vi "Main.vi"() -> ()   [LabVIEW 2026]
uses:
  <vilib>/Instr/_visa.llb/VISA Configure Serial Port (Instr).vi
panel:
  out "SR MODO":enum16{"AUTOMATICO", "MANUAL"}(ring)=enum."MANUAL"
  out "Boton Reset":string
  out "Errores CRC":dbl
  out "Tramas OK":dbl
  out "Estado":string
  out "SALIDA PWM":dbl(graph)
  in  "MODO":bool=TRUE
  in  "RESET":bool
  out "Maquina":T1(ring)
  in  "EMERGENCIA":bool
  in  "PWM":dbl min=0.0 max=100.0
  out "SP Vs ALTURA":cluster{dbl, dbl}(graph)
  out "PING PONG":dbl(slide) scale=0.0..50.0
  out "PID":T2(ring)
  out "error out":errorcluster
  out "Enum":enum16{"DESCONECTADO", "CONECTADO"}(ring)
  out "ESTADO  SYS":enum16{"DETENIDO", "EJECUTANDO", "ERROR"}(ring)
  in  "PARADA":bool
  in  "INICIO":bool
  out "PID":string
  in  "SP":dbl=25.0 min=0.0 max=100.0
  in  "KD":dbl=0.07 min=0.0 max=65535.0
  in  "KI":dbl=0.14 min=0.0 max=65535.0
  in  "KP":dbl=3.9 min=0.0 max=65535.0
  in  "PID":bool
  out "PWM":dbl format="%.2g"
  out "ERROR":dbl format="%.2g"
  out "ALTURA":dbl format="%.2g"
  out "SP":dbl format="%.2f"
  out "array":string[][](array[string])
  out "Procesar":string
  in  "Stop Simulation":bool
  in  "Numeric":u32=115200
  in  "VISA resource name":refnum<visa-resource-name>="COM12"
  out "Iteracion":i32
  # "Sistema Levitador Neumático"
  # "Planta"
  # "Grafico en Tiempo Real"
  # "COMUNICACIÓN"
  # "ESTADO DEL SISTEMA"
  # "Estado :"
  # "Puerto :"
  # "Comunicación :"
  # "Baud :"
  # "Estado PID :"
  # "CONFIGURACIÓN PID"
  # "VARIABLES EN TIEMPO REAL"
  # "KP :"
  # "KI  :"
  # "KD :"
  # "AUTO"
  # "MANUAL"
  # "SP :"
  # "PWM :"
  # "Mensaje a Procesar :"
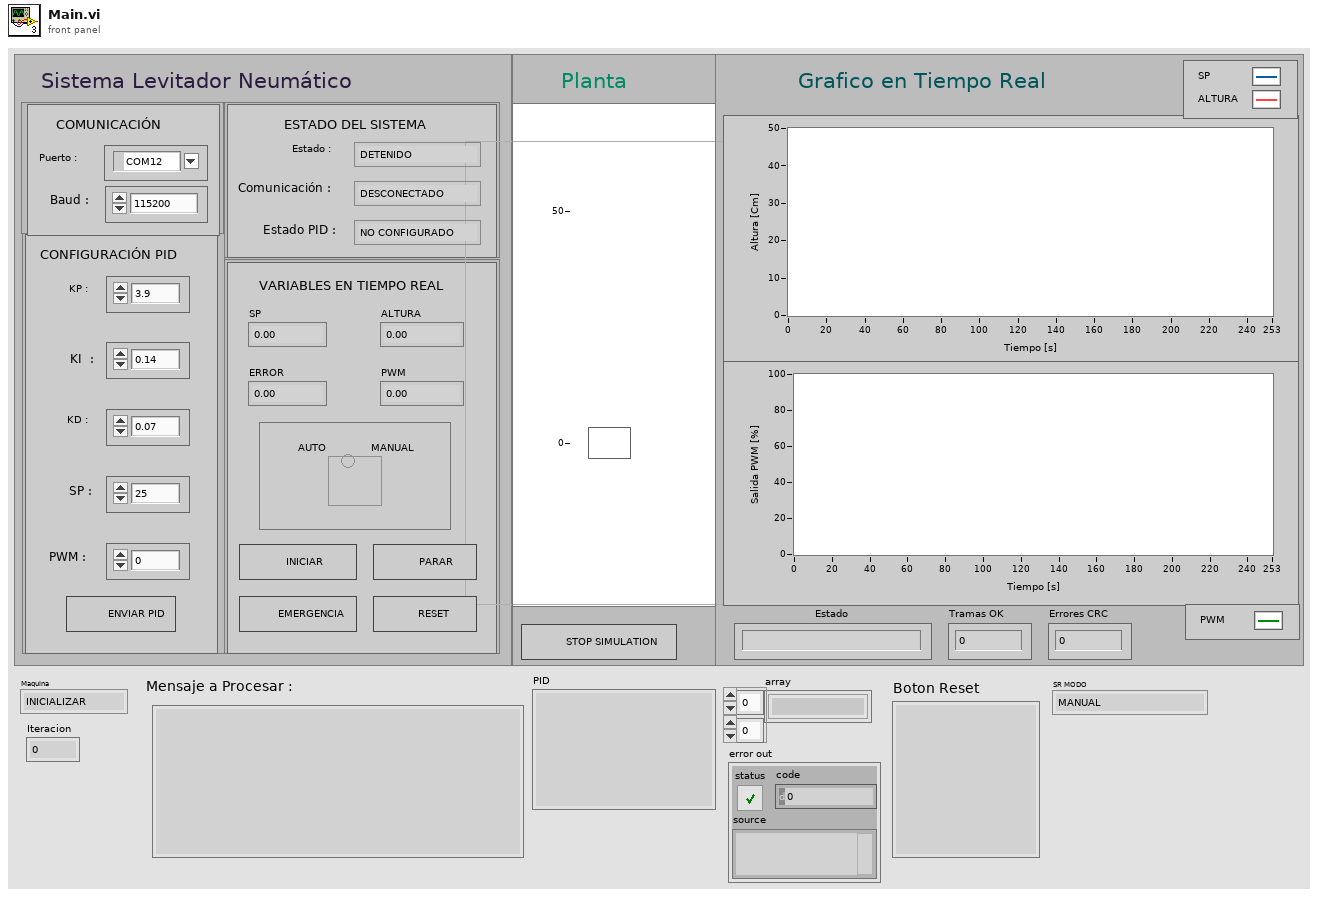
[diagram p1: front panel]
types:
  T1 = enum16{"INICIALIZAR", "ESPERA", "ENVIAR_MODO", "ENVIAR_SP", "ENVIAR_PID", "RECIBIR", "PROCESAR", "ENVIAR_RESET", "ENVIAR_RUN", "ENVIAR_STOP", "ENVIAR_EMERGENCIA_ON", "ENVIAR_EMERGENCIA_OFF", "ERROR", "CERRAR"}
  T2 = enum16{"NO CONFIGURADO", "CONFIGURADO", "AUTOMATICO"}
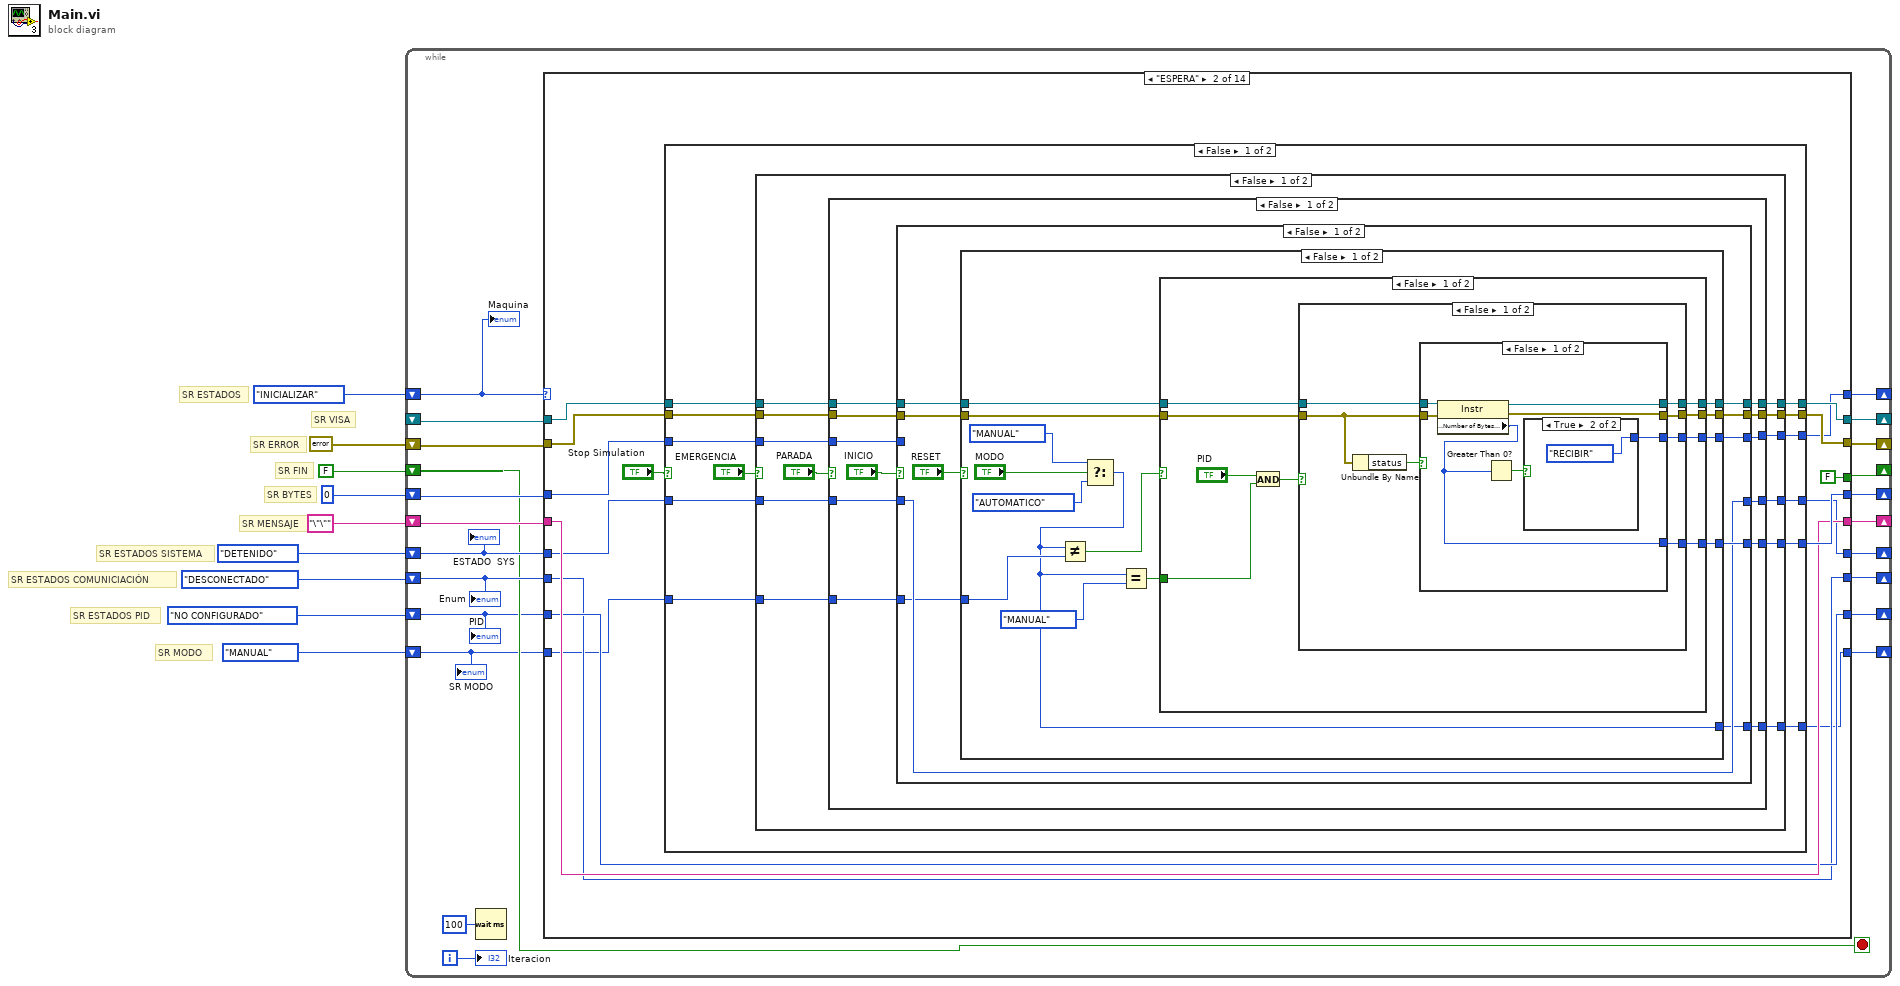
[diagram p0: block diagram]
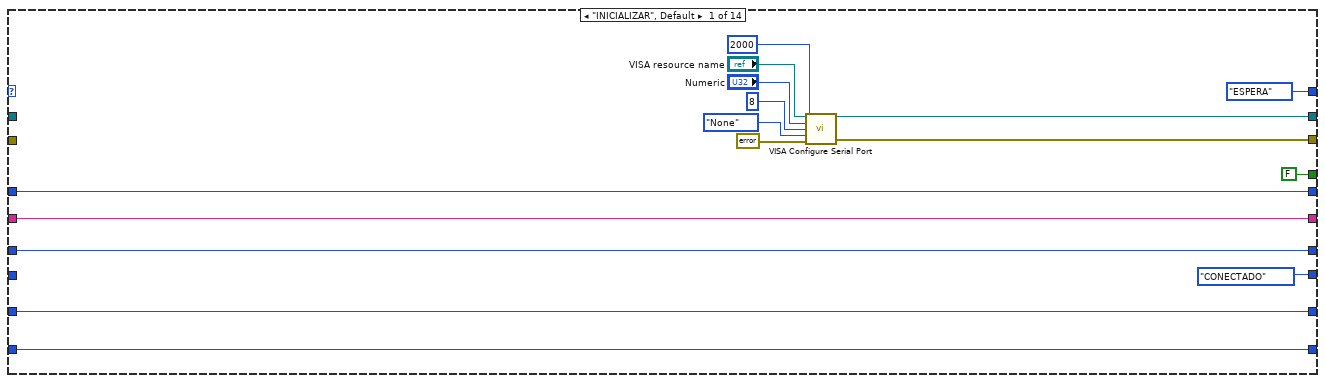
[diagram p2: hidden frame]
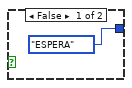
[diagram p3: hidden frame]
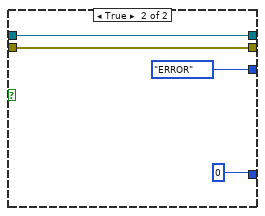
[diagram p4: hidden frame]
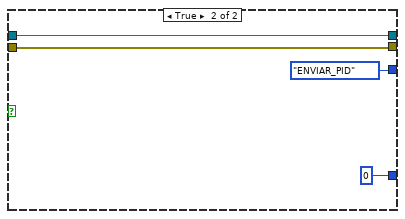
[diagram p5: hidden frame]
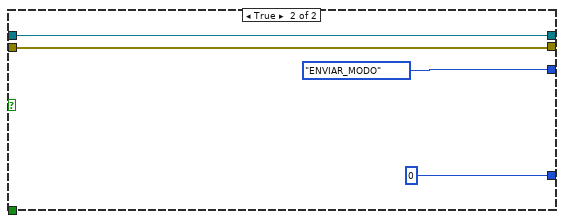
[diagram p6: hidden frame]
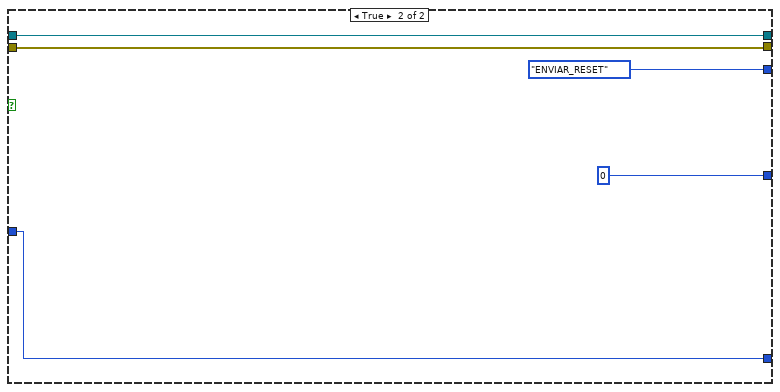
[diagram p7: hidden frame]
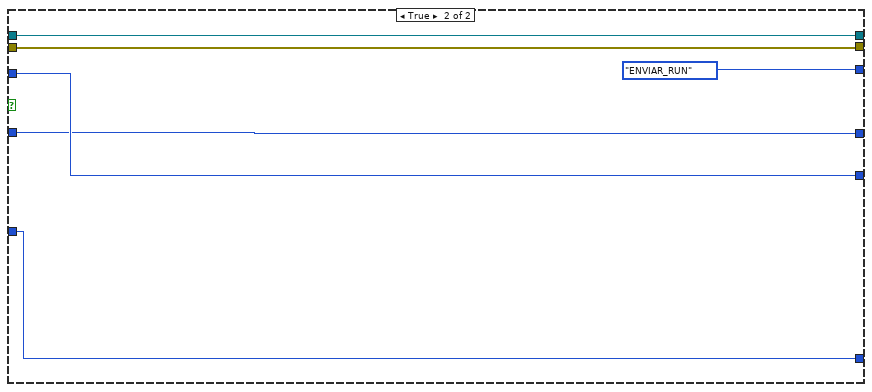
[diagram p8: hidden frame]
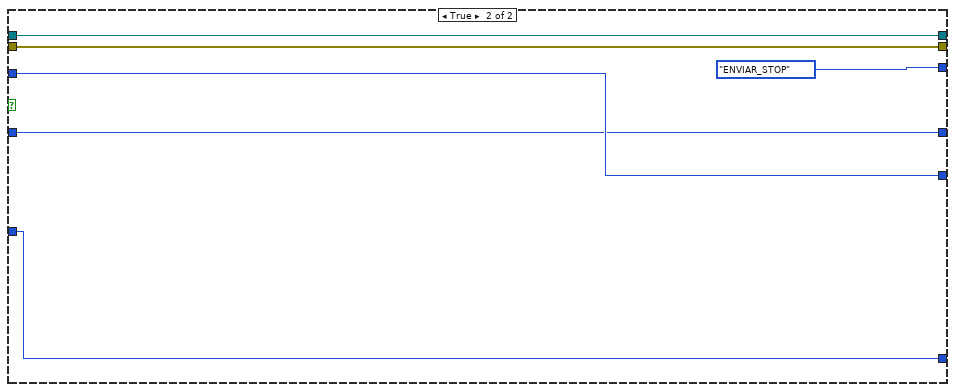
[diagram p9: hidden frame]
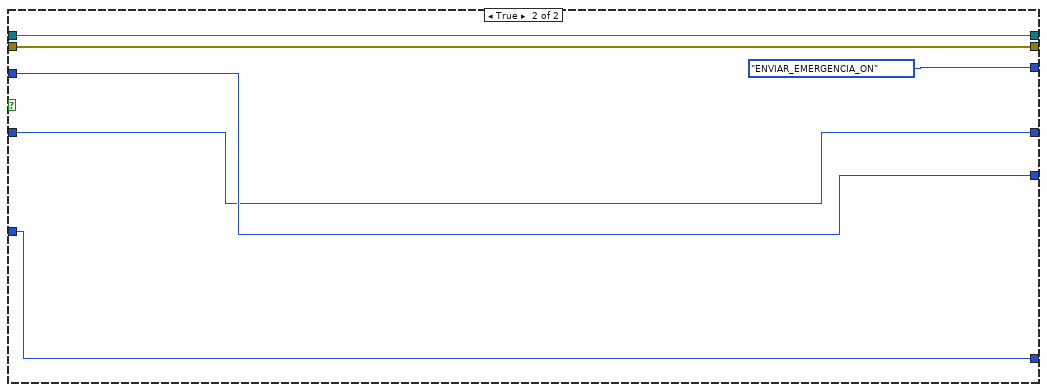
[diagram p10: hidden frame]
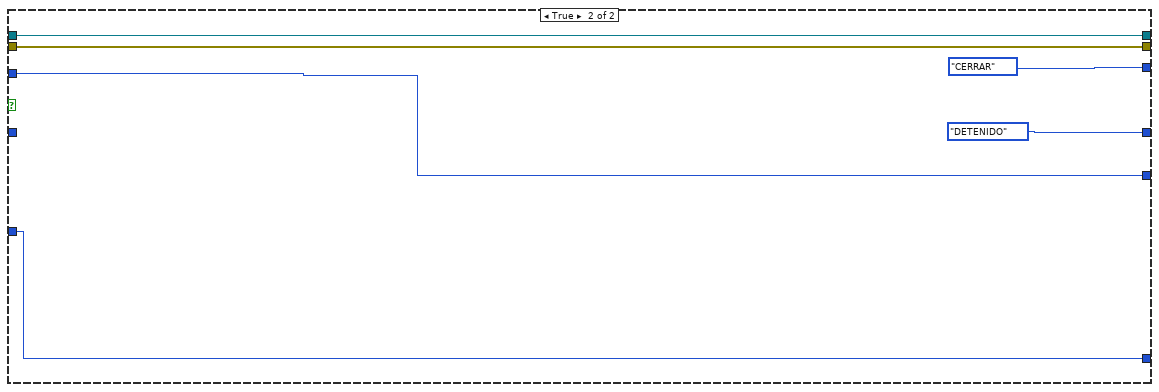
[diagram p11: hidden frame]
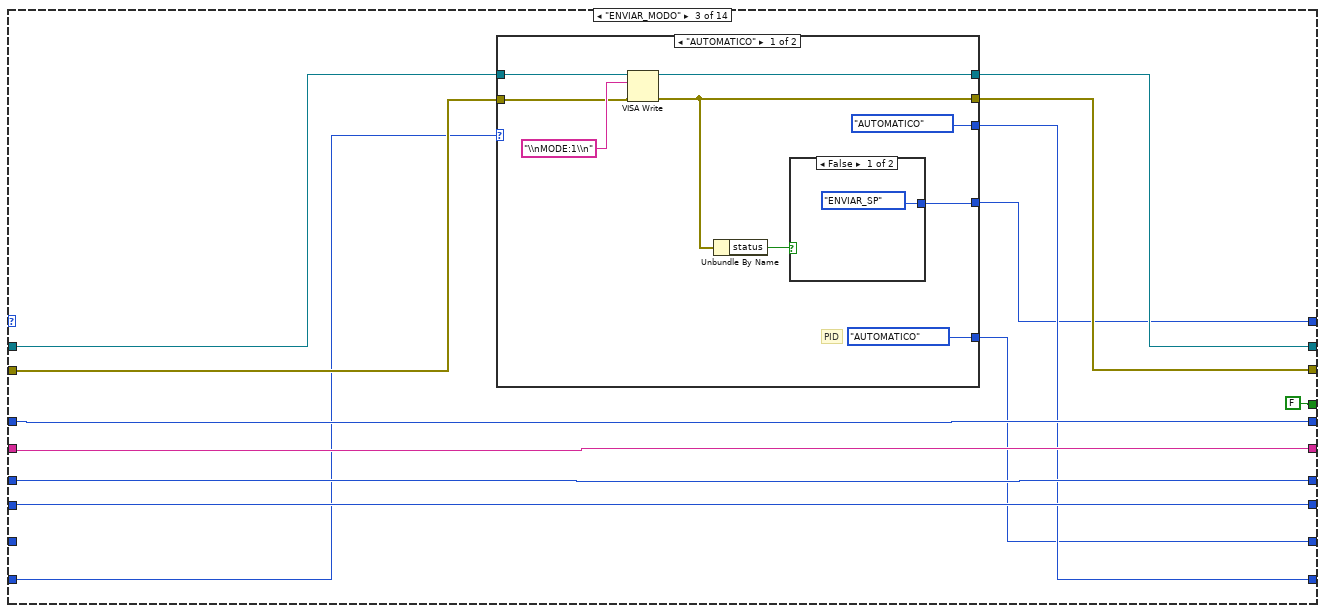
[diagram p12: hidden frame]
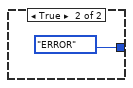
[diagram p13: hidden frame]
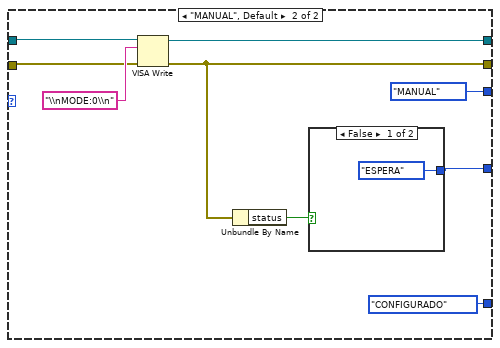
[diagram p14: hidden frame]
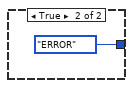
[diagram p15: hidden frame]
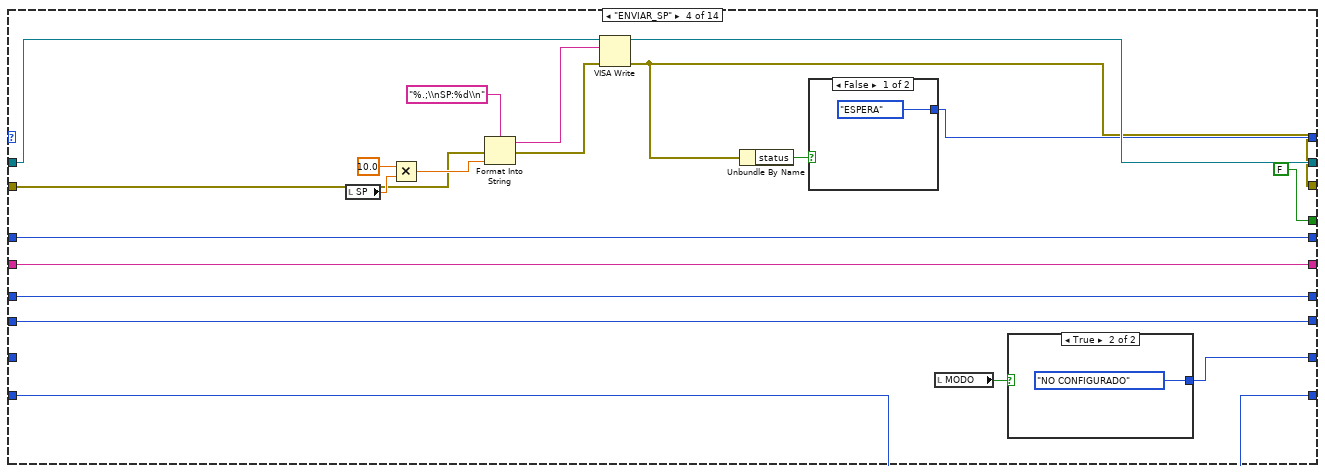
[diagram p16: hidden frame]
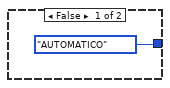
[diagram p17: hidden frame]
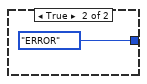
[diagram p18: hidden frame]
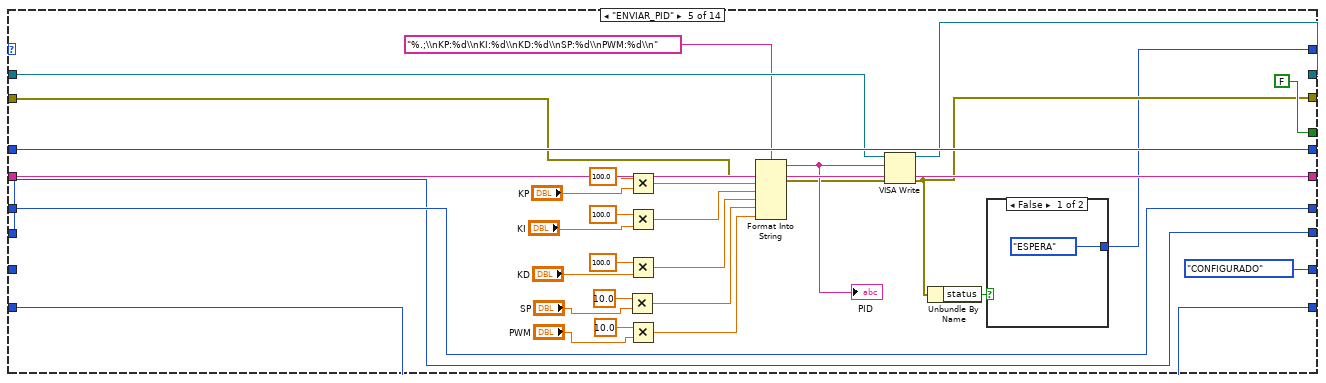
[diagram p19: hidden frame]
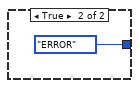
[diagram p20: hidden frame]
diagram:
  # "SR MODO"
  # "SR ESTADOS PID"
  # "SR ESTADOS COMUNICIACIÓN"
  # "SR ESTADOS SISTEMA"
  # "SR MENSAJE"
  # "SR BYTES"
  # "SR FIN"
  # "SR ERROR"
  # "SR ESTADOS"
  # "SR VISA"
  n1 = while {
    shift-right: [w29] -> _
    shift-left: _ -> [w27]
    shift-right: [w28] -> _
    shift-left: errorcluster {"status"=FALSE, "code"=0, "source"=""} ("error out") -> [w26]
    shift-right: [w25] -> _
    shift-left: FALSE -> [w16]
    shift-right: [w24] -> _
    shift-left: u32 0 ("Bytes at Port") -> [w23]
    shift-right: [w22] -> _
    shift-left: "\"\"" -> [w21]
    shift-right: [w17] -> _
    shift-left: enum16{"DETENIDO", "EJECUTANDO", "ERROR"}."DETENIDO" -> [w19]
    shift-right: [w18] -> _
    shift-left: enum16{"DESCONECTADO", "CONECTADO"}."DESCONECTADO" -> [w20]
    shift-right: [w14] -> _
    shift-left: T2."NO CONFIGURADO" -> [w15]
    shift-right: [w12] -> _
    shift-left: T1."INICIALIZAR" -> [w13]
    shift-right: [w10] -> _
    shift-left: enum16{"AUTOMATICO", "MANUAL"}."MANUAL" -> [w11]
    i -> [w31]
    stop <- w16 stop-if-true
    n2 = Wait (ms)(milliseconds to wait=u32 100) -> ()  [unwired: 1 out]
    n3 = case shown="\"ESPERA\"" w13 {
      tunnel: [T1."ESPERA" w48 w191 w229 w268 w286 T1."ESPERA" w382 w401 w415 w433 w449 T1."CERRAR" T1."CERRAR"] -> w12
      tunnel: [w41 w61 w195 w230 w273 w291 w322 w384 w403 w416 w430 w451 w467 w471] -> w29
      tunnel: [w40 w60 w194 w228 w270 w288 w313 w378 w402 w417 w429 w450 w463 w472] -> w28
      tunnel: w27 -> [_ w62 w197 w232 w274 w293 w322 w386 w405 w421 w435 w453 w467 w471]
      tunnel: w26 -> [_ w56 w196 w231 w276 w292 w314 w385 w404 w420 w434 w452 w463 w473]
      tunnel: [FALSE FALSE FALSE FALSE FALSE FALSE FALSE FALSE FALSE FALSE FALSE FALSE FALSE TRUE] -> w25
      tunnel: [w38 w59 w200 w241 w278 w290 w309 w381 w398 w418 w431 w446 w465 w477] -> w24
      tunnel: w23 -> [w38 w58 w200 w241 w278 w290 w309 w381 w398 w418 w431 w446 w465 w477]
      tunnel: [w37 w57 w201 w242 w277 w289 w307 w380 w399 w419 w428 w445 w464 w476] -> w22
      tunnel: w21 -> [w37 w57 w201 w242 w277 _ w307 w380 w399 w419 w428 w445 w464 w476]
      tunnel: w19 -> [w36 w54 w199 w244 w267 w285 w300 w379 _ _ _ w442 w462 _]
      tunnel: w20 -> [_ w51 w198 w240 w251 w283 w298 w377 w395 w411 w427 w443 w459 _]
      tunnel: [enum16{"DESCONECTADO", "CONECTADO"}."CONECTADO" w51 w198 w240 w251 w283 w298 w377 w395 w411 w427 w443 w459 enum16{"DESCONECTADO", "CONECTADO"}."DESCONECTADO"] -> w18
      tunnel: [w36 w55 w199 w244 w267 w285 w300 w379 enum16{"DETENIDO", "EJECUTANDO", "ERROR"}."EJECUTANDO" enum16{"DETENIDO", "EJECUTANDO", "ERROR"}."DETENIDO" enum16{"DETENIDO", "EJECUTANDO", "ERROR"}."DETENIDO" w442 w462 enum16{"DETENIDO", "EJECUTANDO", "ERROR"}."DETENIDO"] -> w17
      tunnel: w15 -> [w35 w52 _ _ _ w284 w299 _ w396 w412 w432 w447 w461 w470]
      tunnel: [w35 w52 w190 w227 T2."CONFIGURADO" w284 w299 T2."NO CONFIGURADO" w396 w412 w432 w447 w461 w470] -> w14
      tunnel: w11 -> [w32 w50 w192 w225 w249 w282 w297 w375 w394 w410 w426 w444 w458 w468]
      tunnel: [w32 w49 w193 w225 w249 w282 w297 w375 w394 w410 w426 w444 w458 w468] -> w10
      frame "INICIALIZAR", Default {
        n4 = call-poly "VISA Configure Serial Port"("VISA resource name"="VISA resource name", "timeout (10sec)"=u32 2000, "baud rate (9600)"="Numeric", "data bits (8)"=u16 8, "parity (0:none)"=enum16{"None", "Odd", "Even", "Mark", "Space"}."None", "error in (no error)"=errorcluster {"status"=FALSE, "code"=0, "source"=""}) -> ("VISA resource name out"=w41:refnum<visa-resource-name>, "error out"=w40:errorcluster)  [unwired: 8 in]
      }
      frame "ESPERA" {
        n5 = case shown="False" "Stop Simulation" {
          tunnel: [w75 T1."CERRAR"] -> w48
          tunnel: w62 -> [w74 w187]
          tunnel: [w73 w187] -> w61
          tunnel: [w72 w186] -> w60
          tunnel: [w71 w189] -> w59
          tunnel: w58 -> [w70 w189]
          tunnel: w56 -> [w69 w186]
          tunnel: [w68 enum16{"DETENIDO", "EJECUTANDO", "ERROR"}."DETENIDO"] -> w55
          tunnel: w54 -> [w67 _]
          tunnel: w50 -> [w65 w184]
          tunnel: [w64 w184] -> w49
          frame False {
            n6 = case shown="False" "EMERGENCIA" {
              tunnel: [w87 T1."ENVIAR_EMERGENCIA_ON"] -> w75
              tunnel: w74 -> [w79 w181]
              tunnel: [w86 w181] -> w73
              tunnel: [w85 w180] -> w72
              tunnel: [w84 w183] -> w71
              tunnel: w70 -> [w83 w183]
              tunnel: w69 -> [w78 w180]
              tunnel: [w81 w182] -> w68
              tunnel: w67 -> [w80 w182]
              tunnel: w65 -> [w77 w178]
              tunnel: [w76 w178] -> w64
              frame False {
                n7 = case shown="False" "PARADA" {
                  tunnel: [w99 T1."ENVIAR_STOP"] -> w87
                  tunnel: w79 -> [w98 w177]
                  tunnel: w78 -> [w97 w176]
                  tunnel: [w96 w177] -> w86
                  tunnel: [w95 w176] -> w85
                  tunnel: [w94 w175] -> w84
                  tunnel: w83 -> [w92 w175]
                  tunnel: [w91 w174] -> w81
                  tunnel: w80 -> [w90 w174]
                  tunnel: w77 -> [w89 w172]
                  tunnel: [w88 w172] -> w76
                  frame False {
                    n8 = case shown="False" "INICIO" {
                      tunnel: [w109 T1."ENVIAR_RUN"] -> w99
                      tunnel: w98 -> [w108 w171]
                      tunnel: w97 -> [w107 w170]
                      tunnel: [w106 w171] -> w96
                      tunnel: [w105 w170] -> w95
                      tunnel: [w104 w169] -> w94
                      tunnel: w92 -> [_ w169]
                      tunnel: [w103 w168] -> w91
                      tunnel: w90 -> [w103 w168]
                      tunnel: w89 -> [w101 w166]
                      tunnel: [w100 w166] -> w88
                      frame False {
                        n9 = case shown="False" "RESET" {
                          tunnel: [w123 T1."ENVIAR_RESET"] -> w109
                          tunnel: w108 -> [w122 w165]
                          tunnel: w107 -> [w121 w164]
                          tunnel: [w120 w165] -> w106
                          tunnel: [w119 w164] -> w105
                          tunnel: [w118 u32 0 ("Bytes at Port")] -> w104
                          tunnel: w101 -> [w113 w161]
                          tunnel: [w110 w161] -> w100
                          frame False {
                            n10 = Select(t=enum16{"AUTOMATICO", "MANUAL"}."MANUAL", s="MODO", f=enum16{"AUTOMATICO", "MANUAL"}."AUTOMATICO") -> (s? t:f=w110:enum16{"AUTOMATICO", "MANUAL"})
                            n11 = Not Equal?(x=w110, y=w113) -> (x != y?=w114:bool)
                            n12 = Equal?(x=w110, y=enum16{"AUTOMATICO", "MANUAL"}."MANUAL") -> (x = y?=w112:bool)
                            n13 = case shown="False" w114 {
                              tunnel: [w132 T1."ENVIAR_MODO"] -> w123
                              tunnel: w122 -> [w131 w160]
                              tunnel: w121 -> [w130 w159]
                              tunnel: [w129 w160] -> w120
                              tunnel: [w128 w159] -> w119
                              tunnel: [w127 u32 0 ("Bytes at Port")] -> w118
                              tunnel: w112 -> [w126 _]
                              frame False {
                                n14 = And(x="PID", y=w126) -> (x .and. y?=w124:bool)
                                n15 = case shown="False" w124 {
                                tunnel: [w139 T1."ENVIAR_PID"] -> w132
                                tunnel: w131 -> [w138 w155]
                                tunnel: w130 -> [w134 w154]
                                tunnel: [w137 w155] -> w129
                                tunnel: [w136 w154] -> w128
                                tunnel: [w135 u32 0 ("Bytes at Port")] -> w127
                                frame False {
                                n16 = Unbundle By Name(w134) -> ("status"=w133:bool)
                                n17 = case shown="False" w133 {
                                tunnel: [w146 T1."ERROR"] -> w139
                                tunnel: w138 -> [w145 w152]
                                tunnel: w134 -> [w144 w151]
                                tunnel: [w143 w152] -> w137
                                tunnel: [w142 w151] -> w136
                                tunnel: [w140 u32 0 ("Bytes at Port")] -> w135
                                frame False {
                                n18 = property class="Instr"(reference=w145, error in=w144) -> (reference out=w143:refnum<visa-resource-name>, error out=w142:errorcluster, "Serial Settings:Number of Bytes at Serial Port"=w140:u32)
                                n19 = Greater Than 0?(x=w140) -> (x > 0?=w141:bool)
                                n20 = case shown="True" w141 {
                                tunnel: [T1."ESPERA" T1."RECIBIR"] -> w146
                                frame False {
                                }
                                frame True {
                                }
                                }
                                }
                                frame True {
                                }
                                }
                                }
                                frame True {
                                }
                                }
                              }
                              frame True {
                              }
                            }
                          }
                          frame True {
                          }
                        }
                      }
                      frame True {
                      }
                    }
                  }
                  frame True {
                  }
                }
              }
              frame True {
              }
            }
          }
          frame True {
          }
        }
      }
      frame "ENVIAR_MODO" {
        n21 = case shown="\"AUTOMATICO\"" w192 {
          tunnel: w197 -> [w209 w221]
          tunnel: w196 -> [w208 w220]
          tunnel: [w207 w218] -> w195
          tunnel: [w206 w219] -> w194
          tunnel: [enum16{"AUTOMATICO", "MANUAL"}."AUTOMATICO" enum16{"AUTOMATICO", "MANUAL"}."MANUAL"] -> w193
          tunnel: [w204 w215] -> w191
          tunnel: [T2."AUTOMATICO" T2."CONFIGURADO"] -> w190
          frame "AUTOMATICO" {
            # "PID"
            n22 = VISA Write(VISA resource name=w209, write buffer="\\nMODE:1\\n", error in (no error)=w208) -> (VISA resource name out=w207:refnum<visa-resource-name>, error out=w206:errorcluster)  [unwired: 1 out]
            n23 = Unbundle By Name(w206) -> ("status"=w210:bool)
            n24 = case shown="False" w210 {
              tunnel: [T1."ENVIAR_SP" T1."ERROR"] -> w204
              frame False {
              }
              frame True {
              }
            }
          }
          frame "MANUAL", Default {
            n25 = VISA Write(VISA resource name=w221, write buffer="\\nMODE:0\\n", error in (no error)=w220) -> (VISA resource name out=w218:refnum<visa-resource-name>, error out=w219:errorcluster)  [unwired: 1 out]
            n26 = Unbundle By Name(w219) -> ("status"=w217:bool)
            n27 = case shown="False" w217 {
              tunnel: [T1."ESPERA" T1."ERROR"] -> w215
              frame False {
              }
              frame True {
              }
            }
          }
        }
      }
      frame "ENVIAR_SP" {
        n28 = local read "SP"() -> (w233:dbl)
        n29 = Multiply(x=10.0, y=w233) -> (x*y=w237:dbl)
        n30 = Format Into String(format string="%.;\\nSP:%d\\n", error in=w231, w237) -> (resulting string=w239:string, error out=w238:errorcluster)  [unwired: 1 in]
        n31 = VISA Write(VISA resource name=w232, write buffer=w239, error in (no error)=w238) -> (VISA resource name out=w230:refnum<visa-resource-name>, error out=w228:errorcluster)  [unwired: 1 out]
        n32 = Unbundle By Name(w228) -> ("status"=w236:bool)
        n33 = case shown="False" w236 {
          tunnel: [T1."ESPERA" T1."ERROR"] -> w229
          frame False {
          }
          frame True {
          }
        }
        n34 = local read "MODO"() -> (w226:bool)
        n35 = case shown="True" w226 {
          tunnel: [T2."AUTOMATICO" T2."NO CONFIGURADO"] -> w227
          frame False {
          }
          frame True {
          }
        }
      }
      frame "ENVIAR_PID" {
        n36 = Multiply(x=10.0, y="SP") -> (x*y=w255:dbl)
        n37 = Multiply(x=100.0, y="KP") -> (x*y=w258:dbl)
        n38 = Multiply(x=100.0, y="KI") -> (x*y=w262:dbl)
        n39 = Multiply(x=100.0, y="KD") -> (x*y=w266:dbl)
        n40 = Multiply(x=10.0, y="PWM") -> (x*y=w252:dbl)
        n41 = Format Into String(format string="%.;\\nKP:%d\\nKI:%d\\nKD:%d\\nSP:%d\\nPWM:%d\\n", error in=w276, w258, w262, w266, w255, w252) -> (resulting string=w275:string, error out=w271:errorcluster)  [unwired: 1 in]
        "PID" <- w275
        n42 = VISA Write(VISA resource name=w274, write buffer=w275, error in (no error)=w271) -> (VISA resource name out=w273:refnum<visa-resource-name>, error out=w270:errorcluster)  [unwired: 1 out]
        n43 = Unbundle By Name(w270) -> ("status"=w269:bool)
        n44 = case shown="False" w269 {
          tunnel: [T1."ESPERA" T1."ERROR"] -> w268
          frame False {
          }
          frame True {
          }
        }
      }
      frame "RECIBIR" {
        n45 = VISA Read(VISA resource name=w293, byte count=w290, error in (no error)=w292) -> (VISA resource name out=w291:refnum<visa-resource-name>, read buffer=w289:string, error out=w288:errorcluster)  [unwired: 1 out]
        n46 = Unbundle By Name(w288) -> ("status"=w287:bool)
        n47 = case shown="False" w287 {
          tunnel: [T1."PROCESAR" T1."ERROR"] -> w286
          frame False {
          }
          frame True {
          }
        }
      }
      frame "PROCESAR" {
        w306 = 0 ("index (row)")
        n48 = Search and Replace String(input string=w307, search string="<", replace string="" ("replace string (\"\")"), error in=w314) -> (result string=w318:string, error out=w317:errorcluster)  [unwired: 4 in, 2 out]
        n49 = Search and Replace String(input string=w318, search string=">", replace string="" ("replace string (\"\")"), error in=w317) -> (result string=w311:string, error out=w313:errorcluster)  [unwired: 4 in, 2 out]
        n50 = Spreadsheet String To Array(delimiter (Tab)=",", format string="%s", spreadsheet string=w311, array type (2D Dbl)="\"\"") -> (array=w301:string[][])
        "array" <- w301
        n51 = Index Array(array=w301, index (row)=w306, index (col)=w306) -> (element=w305:string)
        n52 = Equal?(x="DATA", y=w305) -> (x = y?=w303:bool)
        n53 = case shown="True" w303 {
          tunnel: w301 -> [_ w353]
          frame False {
          }
          frame True {
            w344 = 0 ("index (row)")
            n54 = Index Array(array=w353, index (row) #1=w344, index (col) #1=1 ("index"), index (row) #2=w344, index (col) #2=2 ("index"), index (row) #3=w344, index (col) #3=3 ("index"), index (row) #4=w344, index (col) #4=4 ("index"), index (row) #5=w344, index (col) #5=5 ("disabled index (col)"), index (row) #6=w344, index (col) #6=6 ("disabled index (col)"), index (row) #7=w344, index (col) #7=7 ("disabled index (col)")) -> (element #1=w370:string, element #2=w361:string, element #3=w360:string, element #4=w359:string, element #5=w349:string, element #6=w336:string, element #7=w335:string)
            n55 = Decimal String To Number(string=w349) -> (number=w347:i32)  [unwired: 2 in, 1 out]
            n56 = Index Array(array=string[] ["Sensor OK", "Pelota en el objetivo (± 5 mm)", "PWM saturado", "Integrador saturado", "Timeout de comunicación", "Pelota fuera de rango"], index=w347) -> (element=→"Estado":string)
            n57 = Search and Replace String(input string=w336, search string=".", replace string="," ("replace string (\"\")")) -> (result string=w338:string)  [unwired: 5 in, 3 out]
            n58 = Search and Replace String(input string=w335, search string=".", replace string="," ("replace string (\"\")")) -> (result string=w337:string)  [unwired: 5 in, 3 out]
            n59 = Search and Replace String(input string=w370, search string=".", replace string="," ("replace string (\"\")")) -> (result string=w368:string)  [unwired: 5 in, 3 out]
            n60 = Search and Replace String(input string=w361, search string=".", replace string="," ("replace string (\"\")")) -> (result string=w357:string)  [unwired: 5 in, 3 out]
            n61 = Search and Replace String(input string=w360, search string=".", replace string="," ("replace string (\"\")")) -> (result string=w356:string)  [unwired: 5 in, 3 out]
            n62 = Search and Replace String(input string=w359, search string=".", replace string="," ("replace string (\"\")")) -> (result string=w355:string)  [unwired: 5 in, 3 out]
            n63 = Fract/Exp String To Number(string=w338) -> (number=→"Tramas OK":dbl)  [unwired: 3 in, 1 out]
            n64 = Fract/Exp String To Number(string=w337) -> (number=→"Errores CRC":dbl)  [unwired: 3 in, 1 out]
            n65 = Fract/Exp String To Number(string=w368) -> (number=w351:dbl)  [unwired: 3 in, 1 out]
            n66 = Fract/Exp String To Number(string=w357) -> (number=w330:dbl)  [unwired: 3 in, 1 out]
            n67 = Fract/Exp String To Number(string=w356) -> (number=w327:dbl)  [unwired: 3 in, 1 out]
            n68 = Fract/Exp String To Number(string=w355) -> (number=w324:dbl)  [unwired: 3 in, 1 out]
            n69 = Divide(x=w351, y=10.0) -> (x/y=w332:dbl)
            "SP" <- w332
            n70 = Divide(x=w330, y=10.0) -> (x/y=w329:dbl)
            "ALTURA" <- w329
            "PING PONG" <- w329
            n71 = Divide(x=w327, y=10.0) -> (x/y=→"PWM" →"SALIDA PWM":dbl)
            n72 = Divide(x=w324, y=10.0) -> (x/y=→"ERROR":dbl)
            n73 = Bundle(w332, w329) -> (→"SP Vs ALTURA":cluster{dbl, dbl})  [unwired: 1 in]
          }
        }
        "Procesar" <- w307
      }
      frame "ENVIAR_RESET" {
        w387 = 0.0 ("input 1")
        n74 = Format Into String(format string="%.;\\nKP:%d\\nKI:%d\\nKD:%d\\nSP:%d\\nPWM:%d\\n", error in=w385, w387, w387, w387, w387, w387) -> (resulting string=w391:string, error out=w389:errorcluster)  [unwired: 1 in]
        "Boton Reset" <- w391
        n75 = VISA Write(VISA resource name=w386, write buffer=w391, error in (no error)=w389) -> (VISA resource name out=w384:refnum<visa-resource-name>, error out=w378:errorcluster)  [unwired: 1 out]
        n76 = Unbundle By Name(w378) -> ("status"=w388:bool)
        n77 = case shown="False" w388 {
          tunnel: [T1."ESPERA" T1."ERROR"] -> w382
          frame False {
          }
          frame True {
          }
        }
      }
      frame "ENVIAR_RUN" {
        n78 = VISA Write(VISA resource name=w405, write buffer="\\nEN:1\\n", error in (no error)=w404) -> (VISA resource name out=w403:refnum<visa-resource-name>, error out=w402:errorcluster)  [unwired: 1 out]
        n79 = Unbundle By Name(w402) -> ("status"=w407:bool)
        n80 = case shown="False" w407 {
          tunnel: [T1."ESPERA" T1."ERROR"] -> w401
          frame False {
          }
          frame True {
          }
        }
      }
      frame "ENVIAR_STOP" {
        n81 = VISA Write(VISA resource name=w421, write buffer="\\nEN:0\\n", error in (no error)=w420) -> (VISA resource name out=w416:refnum<visa-resource-name>, error out=w417:errorcluster)  [unwired: 1 out]
        n82 = Unbundle By Name(w417) -> ("status"=w423:bool)
        n83 = case shown="False" w423 {
          tunnel: [T1."ESPERA" T1."ERROR"] -> w415
          frame False {
          }
          frame True {
          }
        }
      }
      frame "ENVIAR_EMERGENCIA_ON" {
        n84 = VISA Write(VISA resource name=w435, write buffer="\\nEMG:1\\n", error in (no error)=w434) -> (VISA resource name out=w430:refnum<visa-resource-name>, error out=w429:errorcluster)  [unwired: 1 out]
        n85 = Unbundle By Name(w429) -> ("status"=w439:bool)
        n86 = case shown="False" w439 {
          tunnel: [T1."RECIBIR" T1."ERROR"] -> w433
          frame False {
          }
          frame True {
          }
        }
      }
      frame "ENVIAR_EMERGENCIA_OFF" {
        n87 = VISA Write(VISA resource name=w453, write buffer="\\nEMG:0\\n", error in (no error)=w452) -> (VISA resource name out=w451:refnum<visa-resource-name>, error out=w450:errorcluster)  [unwired: 1 out]
        n88 = Unbundle By Name(w450) -> ("status"=w455:bool)
        n89 = case shown="False" w455 {
          tunnel: [T1."ESPERA" T1."ERROR"] -> w449
          frame False {
          }
          frame True {
          }
        }
      }
      frame "ERROR" {
        "error out" <- w463
      }
      frame "CERRAR" {
        n90 = VISA Close(VISA resource name=w471, error in (no error)=w473) -> (error out=w472:errorcluster)
      }
    }
    "Iteracion" <- w31
    "ESTADO  SYS" <- w19
    "Enum" <- w20
    "PID" <- w15
    "Maquina" <- w13
    "SR MODO" <- w11
  }
